vi "Query IDN.vi"(8 "error in (no error)":errorcluster, 11 "AUDIX EM1000 in":refnum<class "AUDIX EM1000.lvclass">) -> (0 "error out":errorcluster, 2 "Connected?":bool, 3 "AUDIX EM1000 out":refnum<class "AUDIX EM1000.lvclass">)   [LabVIEW 2023, in "Turn Table and Mast.lvlib" / "AUDIX EM1000.lvclass"]
uses:
  AUDIX EM1000.lvclass
  AUDIX EM1000.lvclass/AUDIX EM1000.ctl
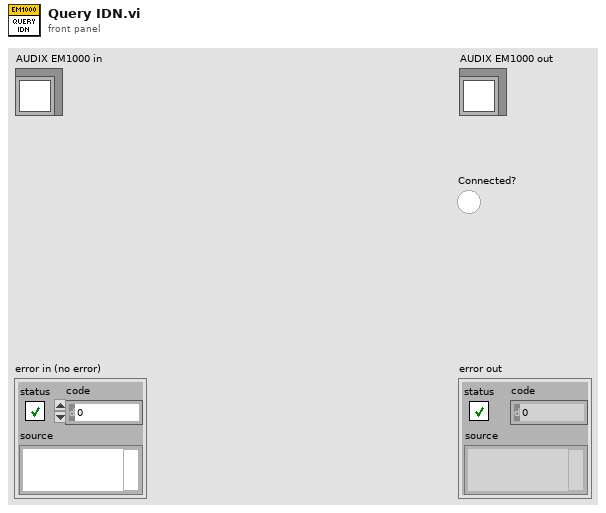
[diagram p1: front panel]
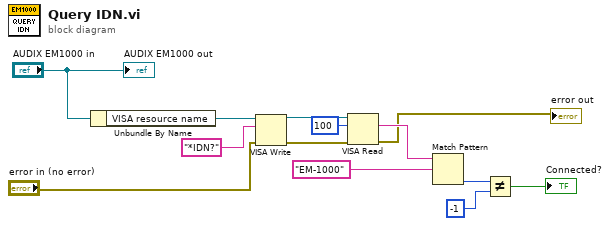
[diagram p0: block diagram]
diagram:
  n1 = Unbundle By Name("AUDIX EM1000 in") -> ("VISA resource name"=w13:refnum<visa-resource-name>)
  n2 = VISA Write(VISA resource name=w13, write buffer="*IDN?", error in (no error)="error in (no error)") -> (VISA resource name out=w11:refnum<visa-resource-name>, error out=w10:errorcluster)  [unwired: 1 out]
  n3 = VISA Read(VISA resource name=w11, byte count=u32 100, error in (no error)=w10) -> (read buffer=w8:string, error out=→"error out":errorcluster)  [unwired: 2 out]
  n4 = Match Pattern(string=w8, regular expression="EM-1000") -> (offset past match=w6:i32)  [unwired: 1 in, 3 out]
  n5 = Not Equal?(x=w6, y=-1) -> (x != y?=→"Connected?":bool)
  "AUDIX EM1000 out" <- "AUDIX EM1000 in"
